vi "Move Clock Wise.vi"(8 "error in (no error)":errorcluster, 11 "CO3000 in":refnum<class "CO3000.lvclass">) -> (0 "error out":errorcluster, 3 "CO3000 out":refnum<class "CO3000.lvclass">)   [LabVIEW 2023, in "Turn Table and Mast.lvlib" / "CO3000.lvclass"]
uses:
  CO3000.lvclass
  CO3000.lvclass/CO3000.ctl
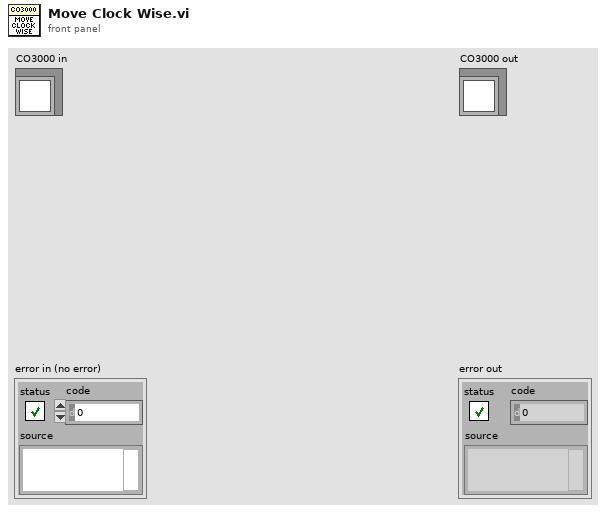
[diagram p1: front panel]
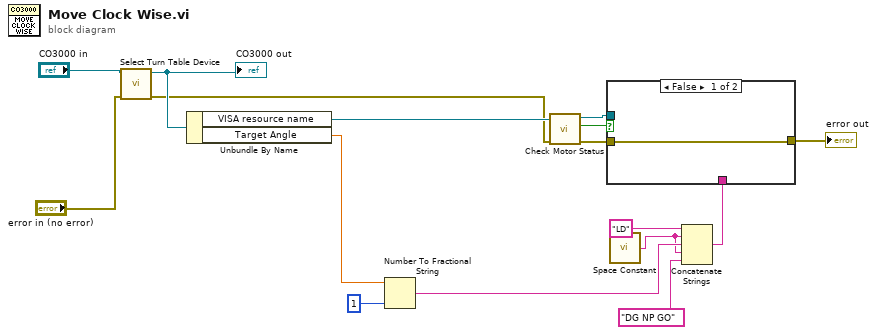
[diagram p0: block diagram]
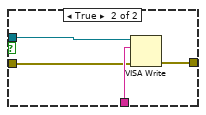
[diagram p2: hidden frame]
diagram:
  n1 = call "Select Turn Table Device.vi"("error in (no error)"="error in (no error)", "CO3000 in"="CO3000 in") -> ("error out"=w2:errorcluster, "CO3000 out"=w4:refnum<class "CO3000.lvclass">)  [unwired: 8 in]
  "CO3000 out" <- w4
  n2 = Unbundle By Name(w4) -> ("VISA resource name"=w16:refnum<visa-resource-name>, "Target Angle"=w14:dbl)
  n3 = Number To Fractional String(number=w14, precision (6)=i16 1) -> (F-format string=w13:string)  [unwired: 2 in]
  n4 = call "Check Motor Status.vi"("error in (no error)"=w2, "VISA Refnum in"=w16) -> ("error out"=w6:errorcluster, "Motor Stop?"=w8:bool, "VISA Refnum out"=w7:refnum<visa-resource-name>)  [unwired: 7 in]
  n5 = call <vilib>:"Space Constant.vi"() -> ("String"=w12:string)
  n6 = Concatenate Strings("LD" ("string"), w12, w13, w12, "DG NP GO" ("string")) -> (w10:string)
  n7 = case shown="False" w8 {
    tunnel: w10 -> [_ w21]
    tunnel: [w17 w20] -> w9
    tunnel: w7 -> [_ w19]
    tunnel: w6 -> [w17 w18]
    frame False {
    }
    frame True {
      n8 = VISA Write(VISA resource name=w19, write buffer=w21, error in (no error)=w18) -> (error out=w20:errorcluster)  [unwired: 2 out]
    }
  }
  "error out" <- w9
